vi "NewPlotStyle (SubVI).vi"(11 "XYGraph in":refnum<vi>) -> (3 "Array":T1(array[cluster]))   [LabVIEW 2017]
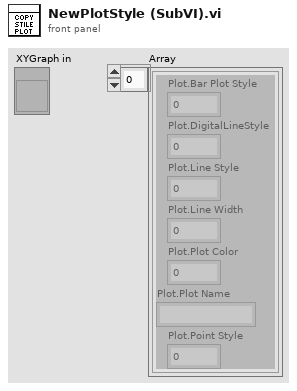
[diagram p1: front panel]
types:
  T1 = cluster{"Plot.Bar Plot Style":u8, "Plot.DigitalLineStyle":u8, "Plot.Line Style":u8, "Plot.Line Width":u8, "Plot.Plot Color":u32, "Plot.Plot Name":string, "Plot.Point Style":u8}[]
  T2 = cluster{"Plot.Bar Plot Style":u8, "Plot.DigitalLineStyle":u8, "Plot.Line Style":u8, "Plot.Line Width":u8, "Plot.Plot Color":u32, "Plot.Plot Name":string, "Plot.Point Style":u8}
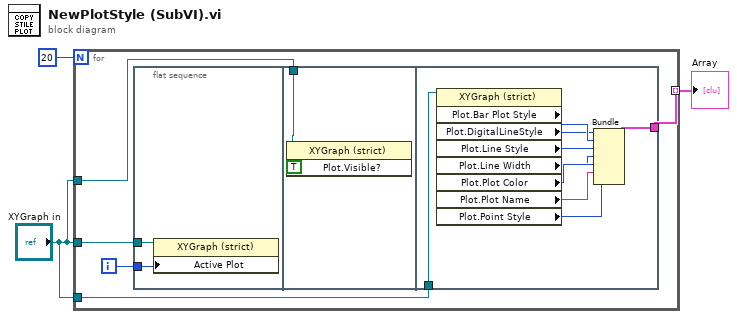
[diagram p0: block diagram]
diagram:
  n1 = for {
    N: 20 -> [_]
    tunnel: [w7] -> w2 mode=indexing
    tunnel: "XYGraph in" -> [w6]
    tunnel: "XYGraph in" -> [w5]
    tunnel: "XYGraph in" -> [w4]
    i -> [w8]
    n2 = flat-sequence {
      tunnel: w8 -> [w10]
      tunnel: w6 -> [w9]
      tunnel: w4 -> [w11]
      tunnel: [w14] -> w7
      tunnel: w5 -> [w13]
      frame #0 {
        n3 = property on="Property Node" class="XYGraph (strict)"(reference=w9, "Active Plot"=w10) -> ()  [unwired: 1 in, 2 out]
      }
      frame #1 {
        n4 = property on="Property Node" class="XYGraph (strict)"(reference=w11, "Plot.Visible?"=TRUE ("Plot.Visible")) -> ()  [unwired: 1 in, 2 out]
      }
      frame #2 {
        n5 = property on="Property Node" class="XYGraph (strict)"(reference=w13) -> ("Plot.Bar Plot Style"=w15:u8, "Plot.DigitalLineStyle"=w16:u8, "Plot.Line Style"=w17:u8, "Plot.Line Width"=w18:u8, "Plot.Plot Color"=w19:u32, "Plot.Plot Name"=w20:string, "Plot.Point Style"=w21:u8)  [unwired: 1 in, 2 out]
        n6 = Bundle("Plot.Bar Plot Style"=w15, "Plot.DigitalLineStyle"=w16, "Plot.Line Style"=w17, "Plot.Line Width"=w18, "Plot.Plot Color"=w19, "Plot.Plot Name"=w20, "Plot.Point Style"=w21) -> (w14:T2)  [unwired: 1 in]
      }
    }
  }
  "Array" <- w2
